vi "Set Save Directory.vi"(8 "error in (no error)":errorcluster, 10 "Path":path, 11 "Abstract DAQ Triggered Actor in":refnum<class "Abstract DAQ Triggered Actor.lvclass">) -> (0 "error out":errorcluster, 3 "Abstract DAQ Triggered Actor out":refnum<class "Abstract DAQ Triggered Actor.lvclass">)   [LabVIEW 2020, in "DAQ Timed SPIM.lvlib" / "Abstract DAQ Triggered Actor.lvlib" / "Abstract DAQ Triggered Actor.lvclass"]
uses:
  Abstract DAQ Triggered Actor.lvclass
  Abstract DAQ Triggered Actor.lvclass/Abstract DAQ Triggered Actor.ctl
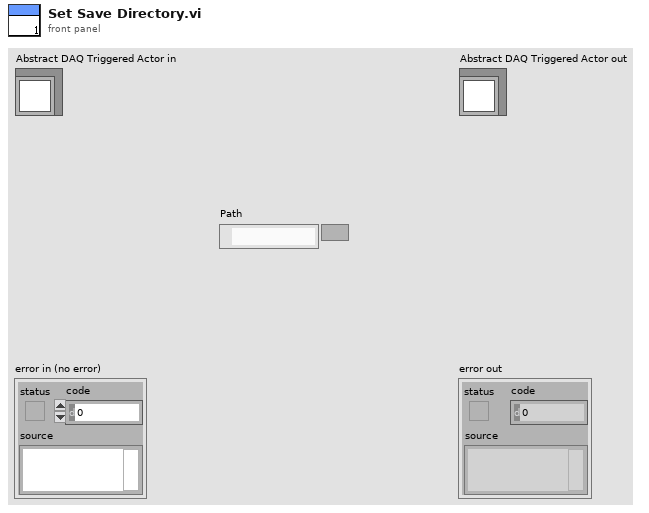
[diagram p1: front panel]
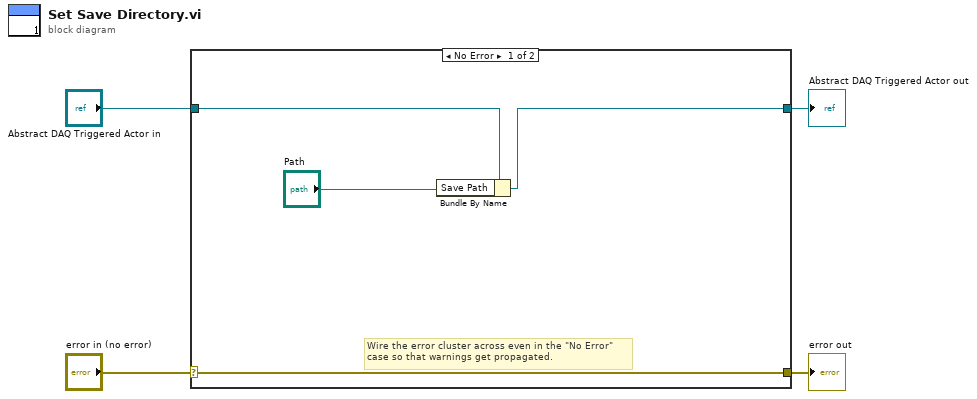
[diagram p0: block diagram]
diagram:
  n1 = case shown="No Error" "error in (no error)" {
    selector: "error in (no error)" -> [w8 w10]
    tunnel: [w8 w10] -> w3
    tunnel: [w5 w9] -> w1
    tunnel: "Abstract DAQ Triggered Actor in" -> [w7 w9]
    frame No Error {
      # "Wire the error cluster across even in the \"No Error\"\ncase so that warnings get propagated."
      n2 = Bundle By Name(cluster=w7, "Save Path"="Path") -> (w5:refnum<class "Abstract DAQ Triggered Actor.lvclass">)
    }
    frame Error {
    }
  }
  "error out" <- w3
  "Abstract DAQ Triggered Actor out" <- w1
